vi "CheckSum_CalcAndSave.vi"(7 "CheckSomeAction":T1=enum."ReadCheckSum", 8 "error in":errorcluster, 10 "CheckSumFile":path, 11 "TestProcedureFile":path) -> (0 "error out":errorcluster, 3 "CheckSumMatched?":bool)   [LabVIEW 2021]
uses:
  Queue Test updator/Controls/Enum_CheckSum_States.ctl
  <vilib>/security/Message Digest/API/Instances/File/SHA-256 File Checksum.vi
  <vilib>/Utility/config.llb/Write Key (String).vi
  <vilib>/Utility/config.llb/Read Key (String).vi
  <vilib>/security/Message Digest/API/NI_Message Digest API.lvlib
  <vilib>/Utility/config.llb/NI_LVConfig.lvlib
panel:
  out "LoadedCheckSum":string
  out "CheckSum":string
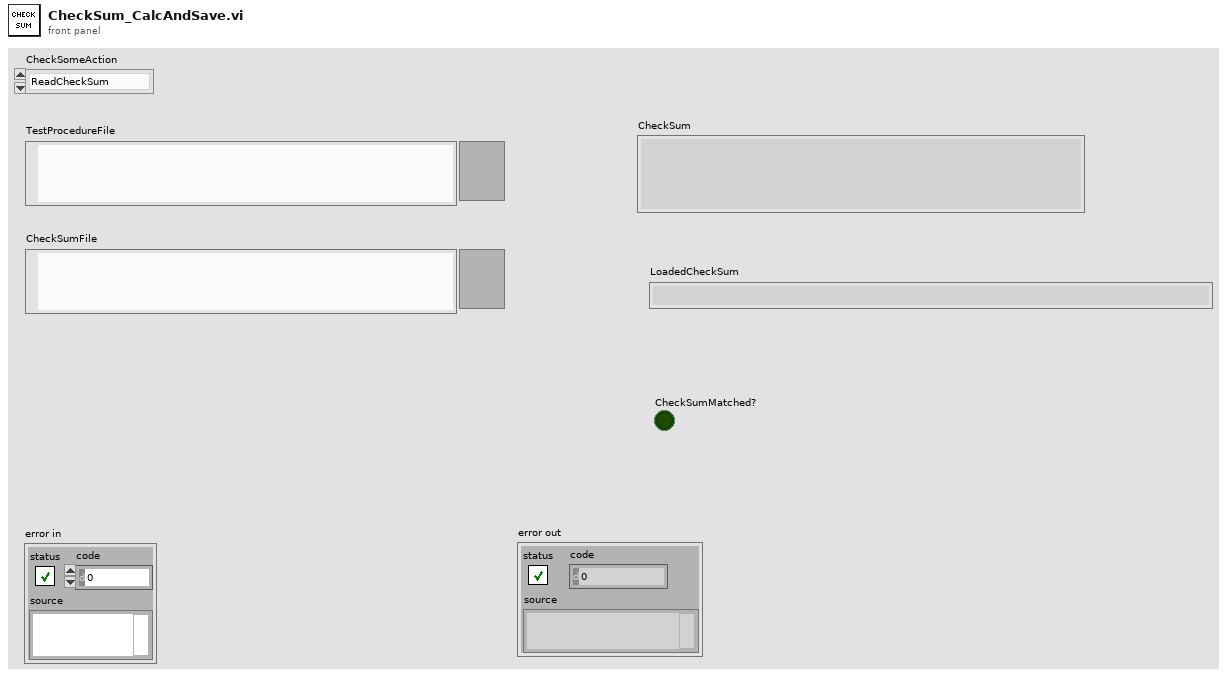
[diagram p1: front panel]
types:
  T1 = typedef "Enum_CheckSum_States.ctl" = enum16{"WriteCheckSum", "ReadCheckSum"}
  T2 = typedef "NI_LVConfig.lvlib/Config Data RefNum.ctl" = refnum<k1>
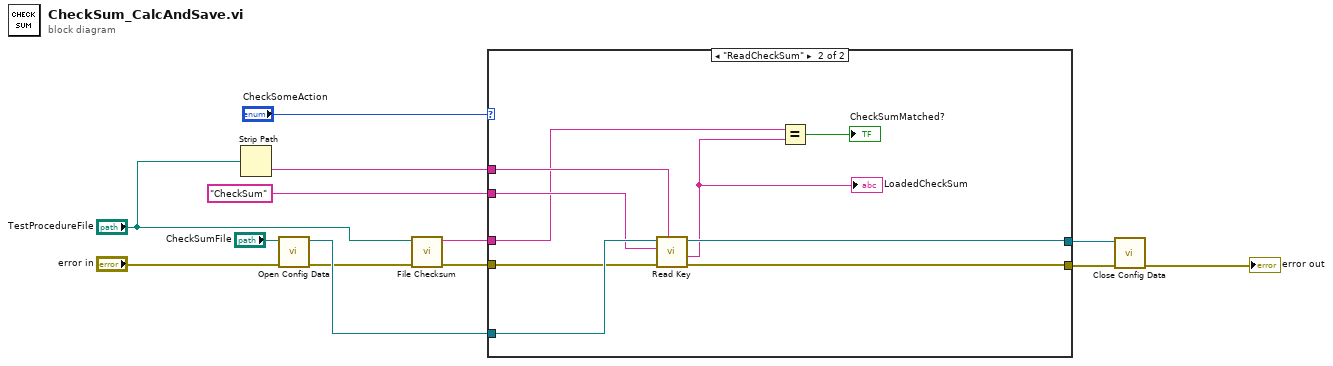
[diagram p0: block diagram]
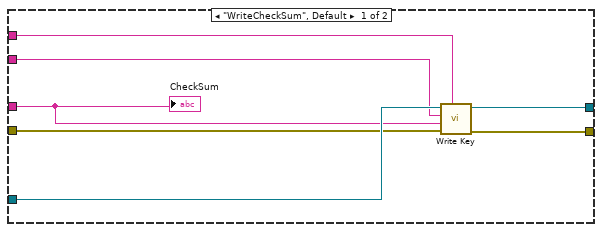
[diagram p2: hidden frame]
diagram:
  n1 = Strip Path(path="TestProcedureFile") -> (name=w6:string)  [unwired: 1 out]
  n2 = call <vilib>:"Open Config Data.vi"("error in (no error)"="error in", "configuration file path"="CheckSumFile") -> ("error out"=w4:errorcluster, "refnum"=w8:T2)  [unwired: 7 in, 1 out]
  n3 = call-poly <vilib>:"File Checksum.vi"("error in"=w4, "path"="TestProcedureFile") -> ("error out"=w3:errorcluster, "digest"=w1:string)  [unwired: 8 in]
  n4 = case shown="\"ReadCheckSum\"" "CheckSomeAction" {
    tunnel: [w20 w24] -> w13
    tunnel: [w19 w25] -> w12
    tunnel: w3 -> [w14 w28]
    tunnel: w8 -> [w18 w29]
    tunnel: w6 -> [w17 w27]
    tunnel: "CheckSum" ("key") -> [w16 w26]
    tunnel: w1 -> [w15 w22]
    frame "WriteCheckSum", Default {
      n5 = call-poly <vilib>:"Write Key.vi"("section"=w17, "error in (no error)"=w14, "value"=w15, "key"=w16, "refnum"=w18) -> ("error out"=w20:errorcluster, "refnum out"=w19:T2)  [unwired: 4 in, 1 out]
      "CheckSum" <- w15
    }
    frame "ReadCheckSum" {
      n6 = call-poly <vilib>:"Read Key.vi"("section"=w27, "error in (no error)"=w28, "key"=w26, "refnum"=w29) -> ("error out"=w24:errorcluster, "value"=w23:string, "refnum out"=w25:T2)  [unwired: 4 in, 1 out]
      "LoadedCheckSum" <- w23
      n7 = Equal?(x=w22, y=w23) -> (x = y?=→"CheckSumMatched?":bool)
    }
  }
  n8 = call <vilib>:"Close Config Data.vi"("error in (no error)"=w13, "refnum"=w12) -> ("error out"=→"error out":errorcluster)  [unwired: 8 in, 1 out]
